vi "Test Client.vi"() -> ()   [LabVIEW 2020]
uses:
  source/Client/Client/Client.lvclass
  source/PV Data/NT Base/NT Base.lvclass
  source/Client/Subscription/Subscription.lvclass
  source/Client/Subscription/Next Value - NT.vi
  source/Client/Client/Put - NT.vi
panel:
  out "Probe":T1
  in  "PV":u16(ring) items=["DEV:BOOL", "DEV:BOOL_ARRAY", "DEV:ENUM", "DEV:FLOAT32", "DEV:FLOAT32_ARRAY", "DEV:FLOAT64", "DEV:FLOAT64_ARRAY", "DEV:INT16", "DEV:INT16_ARRAY", "DEV:INT32", "DEV:INT32_ARRAY", "DEV:INT64", "DEV:INT64_ARRAY", "DEV:INT8", "DEV:INT8_ARRAY", "DEV:STRING", "DEV:STRING_ARRAY", "DEV:UINT16", "DEV:UINT16_ARRAY", "DEV:UINT32", "DEV:UINT32_ARRAY", "DEV:UINT64", "DEV:UINT64_ARRAY", "DEV:UINT8", "DEV:UINT8_ARRAY"]
  in  "Put value":i64
  in  "stop":bool
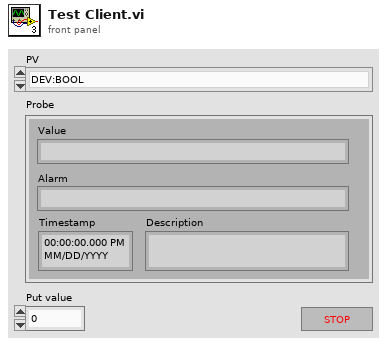
[diagram p1: front panel]
types:
  T1 = cluster{"Timestamp":timestamp, "Value":string, "Description":string, "Alarm":string}
  T2 = typedef "PV Access.lvlib/PV Data.lvlib/Probe.ctl" = cluster{"Timestamp":timestamp, "Value":string, "Description":string, "Alarm":string}
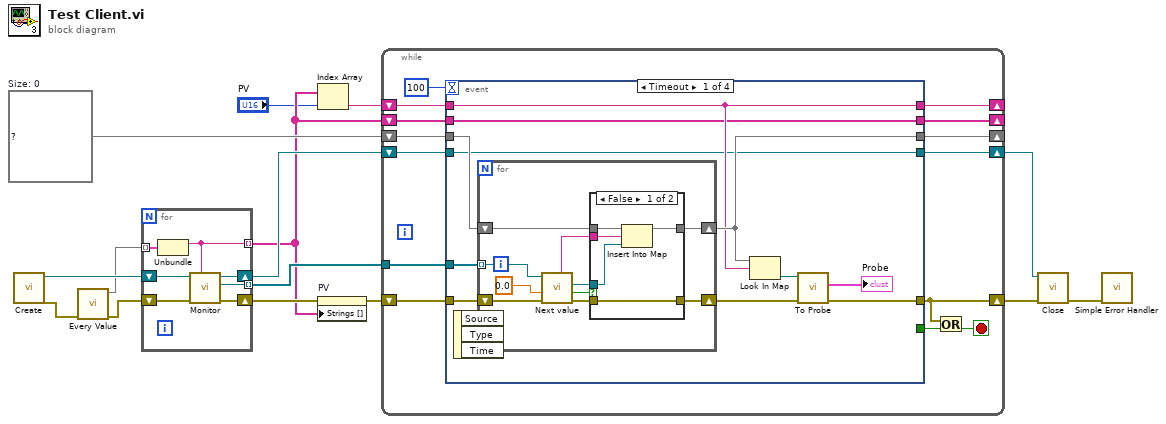
[diagram p0: block diagram]
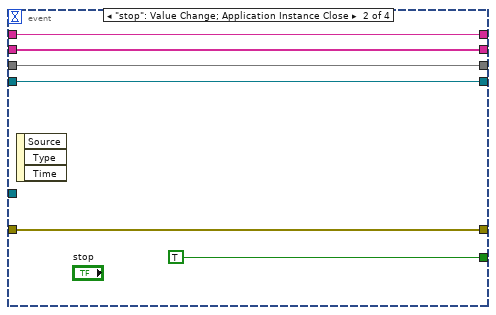
[diagram p3: hidden frame]
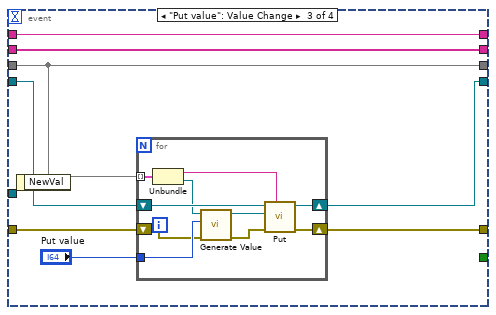
[diagram p4: hidden frame]
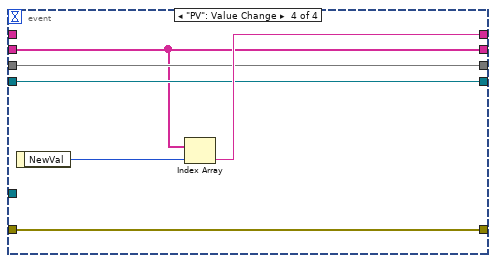
[diagram p5: hidden frame]
diagram:
  w10 = map{string, refnum<class "NT Base.lvclass">} {}  # Size: 0
  n1 = call "Create.vi"() -> ("error out"=w4:errorcluster, "Client out"=w12:refnum<class "Client.lvclass">)  [unwired: 10 in]
  n2 = call "Every Value.vi"("error in (no error)"=w4) -> ("error out"=w3:errorcluster, "values"=w2:map{string, refnum<class "NT Base.lvclass">})  [unwired: 9 in]
  n3 = for {
    shift-right: [w20] -> w11
    shift-left: w12 -> [w22]
    shift-right: [w21] -> w9
    shift-left: w3 -> [w16]
    tunnel: [w19] -> w7 mode=indexing
    tunnel: [w17] -> w5 mode=indexing
    tunnel: w2 -> [w18] mode=indexing
    n4 = Unbundle(w18) -> ("PV name"=w17:string)  [unwired: 1 out]
    n5 = call "Monitor.vi"("PV name"=w17, "error in"=w16, "Client in"=w22) -> ("error out"=w21:errorcluster, "subscription"=w19:refnum<class "Subscription.lvclass">, "Client out"=w20:refnum<class "Client.lvclass">)  [unwired: 6 in]
  }
  n6 = Index Array(array=w5, index="PV") -> (element=w6:string)
  n7 = property on="PV" class="Ring (strict)"(error in=w9, "Strings []"=w5) -> (error out=w8:errorcluster)  [unwired: 1 in, 1 out]
  n8 = while {
    shift-right: [w33] -> w15
    shift-left: w8 -> [w34]
    shift-right: [w32] -> w14
    shift-left: w11 -> [w35]
    shift-right: [w28] -> _
    shift-left: w10 -> [w29]
    shift-right: [w26] -> _
    shift-left: w6 -> [w27]
    shift-right: [w24] -> _
    shift-left: w5 -> [w25]
    tunnel: w7 -> [w30]
    stop <- w36 stop-if-true
    n9 = event shown="[0] Timeout" {
      selector: _ -> [_ _ _ _]
      dyn-events: _ -> [_ _ _ _]
      timeout: 100 -> [_ _ _ _]
      tunnel: w35 -> [w42 w68 w78 w91]
      tunnel: w34 -> [w47 w69 w77 w93]
      tunnel: [w37 w69 w76 w93] -> w33
      tunnel: [w42 w68 w75 w91] -> w32
      tunnel: [_ TRUE ("stop") _ _] -> w31
      tunnel: w30 -> [w46 _ _ _]
      tunnel: w29 -> [w45 w67 w73 w92]
      tunnel: [w44 w67 w73 w92] -> w28
      tunnel: w27 -> [w43 w65 w72 _]
      tunnel: [w43 w65 w72 w94] -> w26
      tunnel: w25 -> [w41 w66 w71 w90]
      tunnel: [w41 w66 w71 w90] -> w24
      event Timeout {
        n10 = event-data() -> ()  [unwired: 1 in, 3 out]
        n11 = for {
          shift-right: [w51] -> w39
          shift-left: w47 -> [w57]
          tunnel: w46 -> [w49] mode=indexing
          shift-right: [w53] -> w44
          shift-left: w45 -> [w54]
          n12 = call-poly "Next value.vi"("error in (no error)"=w57, "timeout"=dbl[unit] 0.0, "Subscription in"=w49) -> ("error out"=w52:errorcluster, "timed out?"=w56:bool, "value"=w55:refnum<class "NT Base.lvclass">, "PV name"=w48:string)  [unwired: 4 in, 1 out]
          n13 = case shown="False" w56 {
            tunnel: w55 -> [w58 _]
            tunnel: w54 -> [w62 w64]
            tunnel: [w61 w64] -> w53
            tunnel: w52 -> [w60 w63]
            tunnel: [w60 w63] -> w51
            tunnel: w48 -> [w59 _]
            frame False {
              n14 = Insert Into Map(map in=w62, key=w59, value=w58) -> (map out=w61:map{string, refnum<class "NT Base.lvclass">})  [unwired: 2 out]
            }
            frame True {
            }
          }
        }
        n15 = Look In Map(map=w44, key=w43) -> (value=w40:refnum<class "NT Base.lvclass">)  [unwired: 1 in, 1 out]
        n16 = call-dynamic "To Probe.vi"("error in (no error)"=w39, "Is Probeable in"=w40) -> ("error out"=w37:errorcluster, "Probe"=→"Probe":T2)  [unwired: 7 in, 1 out]
      }
      event "stop": Value Change; Application Instance Close {
        n17 = event-data() -> ()  [unwired: 1 in, 3 out]
      }
      event "Put value": Value Change {
        n18 = event-data() -> ()  [unwired: 1 in, 1 out]
        n19 = for {
          shift-right: [w88] -> w76
          shift-left: w77 -> [w80]
          tunnel: "Put value" -> [w85]
          tunnel: w73 -> [w82] mode=indexing
          shift-right: [w87] -> w75
          shift-left: w78 -> [w86]
          n20 = Unbundle(w82) -> (w83:string, "Value.lvlib:NTBase.lvclass"=w79:refnum<class "NT Base.lvclass">)
          n21 = call "Generate Value.vi"("error in (no error)"=w80, "base value"=w85, "value in"=w79) -> ("error out"=w81:errorcluster, "value out"=w84:refnum<class "NT Base.lvclass">)  [unwired: 7 in]
          n22 = call-poly "Put.vi"("PV name"=w83, "error in (no error)"=w81, "value in"=w84, "Client in"=w86) -> ("error out"=w88:errorcluster, "Client out"=w87:refnum<class "Client.lvclass">)  [unwired: 4 in, 2 out]
        }
      }
      event "PV": Value Change {
        n23 = event-data() -> ("NewVal"=w89:u16)  [unwired: 1 in]
        n24 = Index Array(array=w90, index=w89) -> (element=w94:string)
      }
    }
    n25 = Or(x=w33, y=w31) -> (x .or. y?=w36:bool)
  }
  n26 = call "Close.vi"("error in (no error)"=w15, "Client in"=w14) -> ("error out"=w13:errorcluster)  [unwired: 9 in]
  n27 = call <vilib>:"Simple Error Handler.vi"("error in (no error)"=w13) -> ()  [unwired: 4 in, 5 out]
